vi "MODBUSDATOS.vi"() -> ()   [LabVIEW 2023]
uses:
  <vilib>/Modbus/master/Create Master Instance (TCP).vi
  <vilib>/Modbus/master/Modbus Master.lvclass
panel:
  out "muestreo":u32
  in  "address":string="192.168.1.6"
  out "Waveform Chart":dbl(graph)
  out "FLUJO":dbl(knob) scale=0.0..10.0
  out "NIVEL":dbl(slide) scale=0.0..10.0
  in  "Vaciado":u16(slide) scale=0.0..100.0
  in  "Llenado":u16(slide) scale=0.0..100.0
  in  "stop":bool
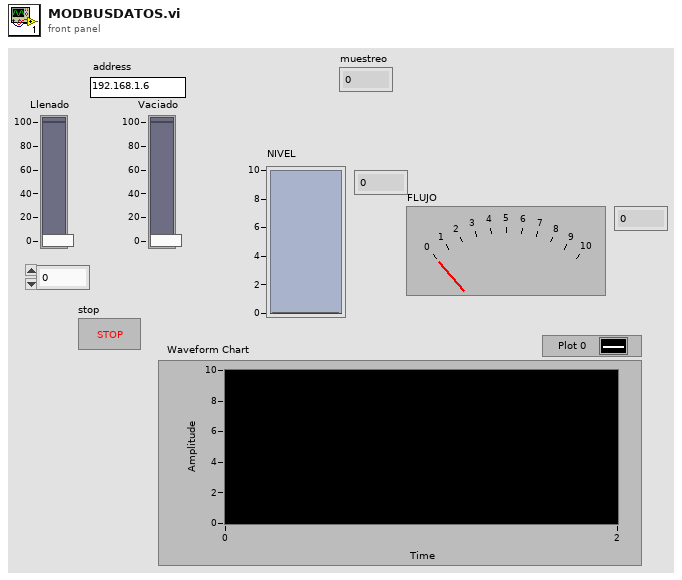
[diagram p1: front panel]
types:
  T1 = enum16{"open", "replace", "create", "open or create", "replace or create", "replace or create with confirmation"}
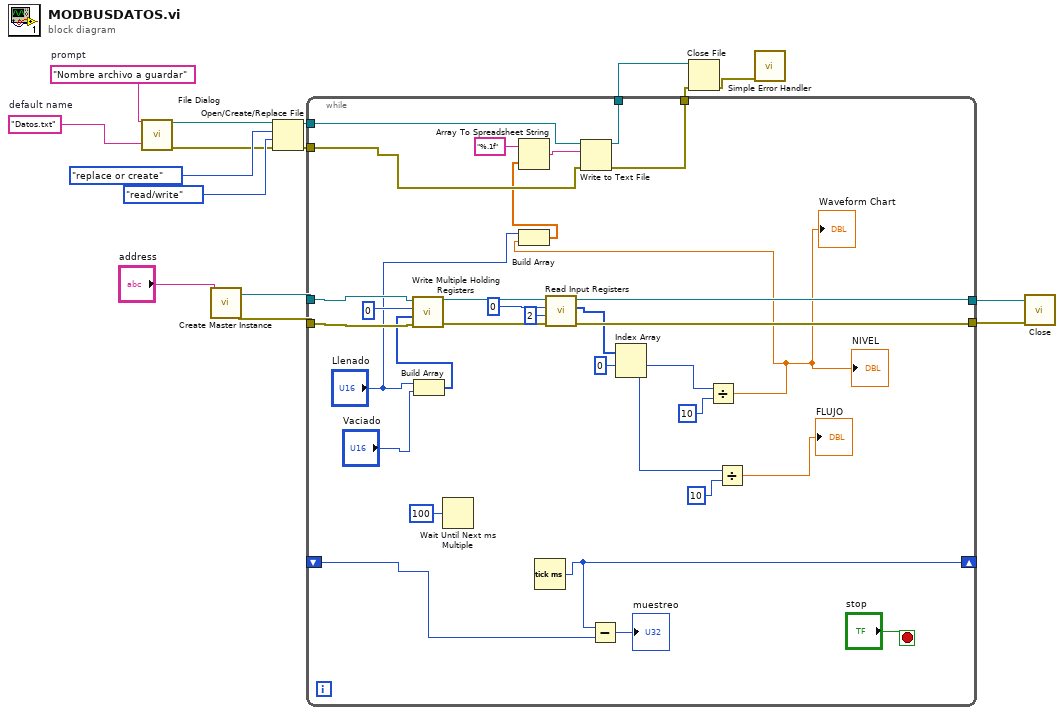
[diagram p0: block diagram]
diagram:
  w12 = "Datos.txt"  # default name
  w7 = "Nombre archivo a guardar"  # prompt
  n1 = call "File Dialog"("prompt"=w7, "pattern (all files)"=w12) -> ("selected path"=w9:path, "error out"=w8:errorcluster)  [unwired: 10 in, 2 out]
  n2 = call-poly <vilib>:"Create Master Instance.vi"("address"="address") -> ("error out"=w15:errorcluster, "TCP master instance"=w16:refnum<class "Modbus Master.lvclass">)  [unwired: 9 in]
  n3 = Open/Create/Replace File(file path (use dialog)=w9, error in=w8, operation (0:open)=T1."replace or create", access (0:read/write)=enum16{"read/write", "read-only", "write-only"}."read/write") -> (refnum out=w6:refnum<file>, error out=w5:errorcluster)  [unwired: 2 in, 1 out]
  n4 = while {
    tunnel: w16 -> [w47]
    tunnel: w15 -> [w45]
    tunnel: [w38] -> w14
    tunnel: [w37] -> w13
    tunnel: w6 -> [w27]
    tunnel: w5 -> [w26]
    tunnel: [w25] -> w3
    tunnel: [w24] -> w2
    shift-right: [w19] -> _
    shift-left: _ -> [w22]
    stop <- "stop" stop-if-true
    n5 = Build Array("Llenado", "Vaciado") -> (w43:u16[])
    n6 = call-dynamic "Write Multiple Holding Registers.vi"("error in (no error)"=w45, "holding register values"=w43, "starting address"=u16 0, "Modbus master in"=w47) -> ("error out"=w41:errorcluster, "Modbus master out"=w42:refnum<class "Modbus Master.lvclass">)  [unwired: 6 in]
    n7 = Wait Until Next ms Multiple(millisecond multiple=u32 100) -> ()  [unwired: 1 out]
    n8 = Tick Count (ms)() -> (millisecond timer value=w19:u32)
    n9 = call-dynamic "Read Input Registers.vi"("error in (no error)"=w41, "number of input registers"=u16 2, "starting address"=u16 0, "Modbus master in"=w42) -> ("error out"=w37:errorcluster, "register values"=w36:u16[], "Modbus master out"=w38:refnum<class "Modbus Master.lvclass">)  [unwired: 5 in]
    n10 = Subtract(x=w19, y=w22) -> (x-y=→"muestreo":u32)
    n11 = Index Array(array=w36, index #1=0 ("index")) -> (element #1=w34:u16, element #2=w31:u16)  [unwired: 1 in]
    n12 = Divide(x=w34, y=u16 10) -> (x/y=w18:dbl)
    "NIVEL" <- w18
    "Waveform Chart" <- w18
    n13 = Build Array("Llenado", w18) -> (w23:dbl[])
    n14 = Array To Spreadsheet String(array=w23, 3:"%.1f") -> (spreadsheet string=w29:string)  [unwired: 1 in]
    n15 = Write to Text File(file (use dialog)=w27, text=w29, error in=w26) -> (refnum out=w24:refnum<file>, error out=w25:errorcluster)  [unwired: 1 in, 1 out]
    n16 = Divide(x=w31, y=u16 10) -> (x/y=→"FLUJO":dbl)
  }
  n17 = Close File(refnum=w2, error in=w3) -> (error out=w4:errorcluster)  [unwired: 1 out]
  n18 = call <vilib>:"Simple Error Handler.vi"("error in (no error)"=w4) -> ()  [unwired: 4 in, 5 out]
  n19 = call-dynamic "Close.vi"("error in (no error)"=w13, "Modbus master in"=w14) -> ()  [unwired: 9 in, 1 out]
